vi "DB Init.vi"(8 "error in (no error)":errorcluster, 11 "DB Path":path) -> (0 "error out":errorcluster, 3 "Connection":refnum<class "Connection.lvclass">)   [LabVIEW 2026]
uses:
  <vilib>/drjdpowell/SQLite Library/SQL Connection/Connection.lvclass
  <vilib>/drjdpowell/SQLite Library/SQL Connection/Open (path).vi
  <vilib>/drjdpowell/SQLite Library/SQL Connection/Open (string).vi
  <vilib>/AdvancedString/Path To Command Line String.vi
  <vilib>/drjdpowell/SQLite Library/SQL Connection/Execute SQL (No results).vi
  <vilib>/drjdpowell/SQLite Library/SQLite.lvlib
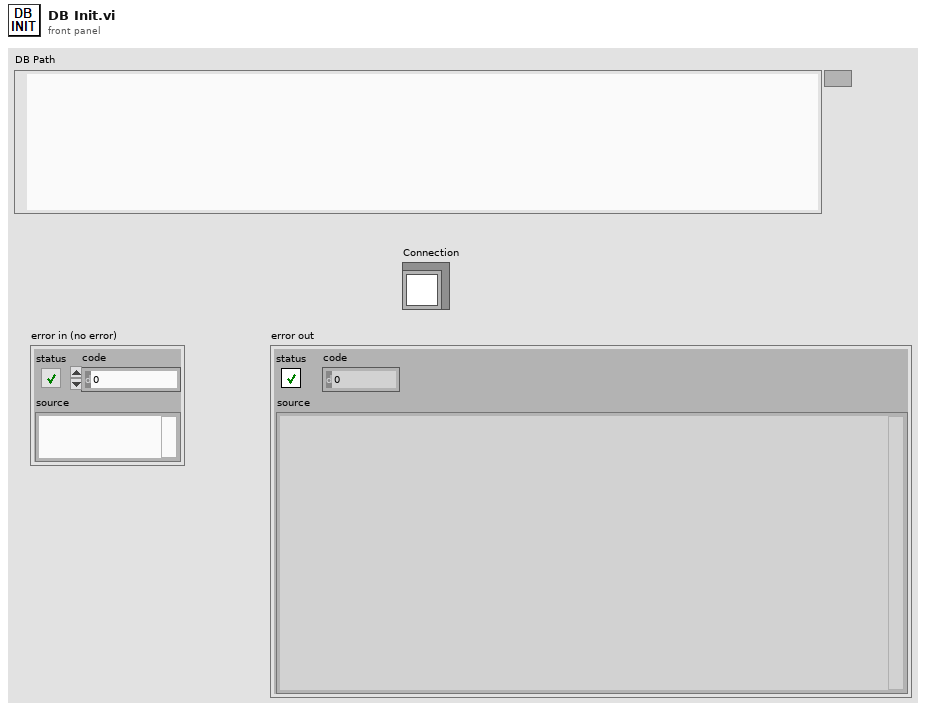
[diagram p1: front panel]
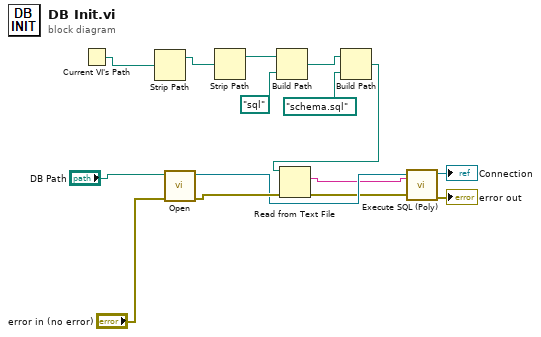
[diagram p0: block diagram]
diagram:
  n1 = Current VI's Path() -> (path=w14:path)
  n2 = Strip Path(path=w14) -> (stripped path=w13:path)  [unwired: 1 out]
  n3 = call-poly <vilib>:"Open.vi"("error in (no error)"="error in (no error)", "db file"="DB Path") -> ("error out"=w7:errorcluster, "SQLite Connection"=w6:refnum<class "Connection.lvclass">)  [unwired: 8 in]
  n4 = Strip Path(path=w13) -> (stripped path=w11:path)  [unwired: 1 out]
  n5 = Build Path(base path=w11, name or relative path=path "sql") -> (appended path=w9:path)
  n6 = Build Path(base path=w9, name or relative path=path "schema.sql") -> (appended path=w8:path)
  n7 = Read from Text File(file (use dialog)=w8, error in=w7) -> (text=w5:string, error out=w4:errorcluster)  [unwired: 2 in, 2 out]
  n8 = call-poly <vilib>:"Execute SQL (Poly).vi"("error in (no error)"=w4, "SQL"=w5, "SQLite Connection in"=w6) -> ("error out"=→"error out":errorcluster, "SQLite Connection"=→"Connection":refnum<class "Connection.lvclass">)  [unwired: 7 in]
